vi "Parse Auto.vi"(8 "Command Info In":T1, 10 "Synchronization":enum16{"Start", "Wait"}(ring)=enum."Wait", 11 "Name":string) -> (0 "Command Info Out":T1)   [LabVIEW 2025]
uses:
  <vilib>/Rock Robotics/WPI/Framework/Command Status Info.ctl
  <vilib>/Rock Robotics/WPI/Framework/Completion Status.ctl
  <vilib>/Rock Robotics/WPI/Framework/Completion Notifier.ctl
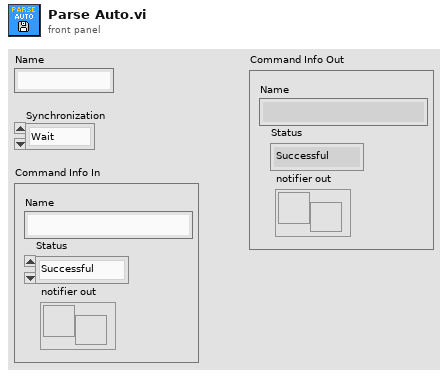
[diagram p1: front panel]
types:
  T1 = typedef "Command Status Info.ctl" = cluster{"Name":string, "Status":T2, "notifier out":T3}
  T2 = typedef "Completion Status.ctl" = enum16{"Successful", "Aborted", "Incomplete"}
  T3 = typedef "Completion Notifier.ctl" = refnum<notifier>
  T4 = typedef "Single Cmd Info NI-LV-Dialog Reference 20261109-211044-511.ctl" = cluster{"Name":string, "CPTM.DataType":variant, "All Control Values Variant":cluster{"Name":string, "Variant Data":variant}[], "icon full":T5, "icon scaled":T5, "Path":path, "Subsystem Color":u32}
  T5 = typedef "imagedata.ctl" = cluster{"image type":i32, "image depth":i32, "image":u8[], "mask":u8[], "colors":u32[], "Rectangle":cluster{"left":i16, "top":i16, "right":i16, "bottom":i16}}
  T6 = typedef "Trajectory Data.ctl" = cluster{"Segment Name":string, "Type":T7, "Traj Pos Points":cluster{"x":dbl, "y":dbl, "th":dbl}[], "Traj Vel Points":cluster{"V":dbl, "Omega":dbl, "V vector":cluster{"y":dbl, "x":dbl}}[], "Accel Index":i32, "Decel Index":i32}[]
  T7 = typedef "Segment Type.ctl" = enum16{"Accel Straight", "Const Straight", "Blend", "Circle", "Bezier"}
  T8 = cluster{"Commands out":cluster{"Time (s)":dbl, T4, bool}[], "Zero V":bool, "Trajectory Data":T6, "Reversals":cluster{"Robot Backwards":bool, "Reverse Path":bool}, "Points out":cluster{"x":dbl, "y":dbl, "th":dbl}[]}
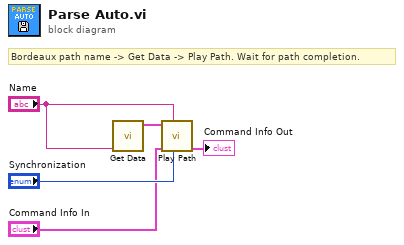
[diagram p0: block diagram]
diagram:
  # "Bordeaux path name -> Get Data -> Play Path. Wait for path completion."
  n1 = call "Get Data.vi"("Name"="Name") -> ("Auto"=w2:T8)  [unwired: 10 in]
  n2 = call "Play Path.vi"("Synchronization"="Synchronization", "Description"="Name", "Command Info In"="Command Info In", "Auto Data"=w2) -> ("Command Info Out"=→"Command Info Out":T1)  [unwired: 7 in]
